vi "Measurement UI.vi"() -> ()   [LabVIEW 2021, in "Line Regulation_PMIC.lvlib"]
uses:
  Line Regulation_PMIC.lvlib
panel:
  in  "MeasGraphs":T1(tab)
  out "LineRegulationGraph(V/V)":T2(graph)
  out "LineRegulationGraph(%)":T3(graph)
  out "Maximum load voltage deviation":dbl
  out "Minimum load voltage deviation":dbl
  out "Maximum load voltage":dbl
  out "Minimum load voltage":dbl
  out "Load voltage deviation":dbl[](array[numeric])
  out "Load voltages":dbl[](array[numeric])
  out "Source voltages":dbl[](array[numeric])
  in  "Source resource name":string caption="RESOURCE NAME"
  in  "Load resource name":string caption="RESOURCE NAME"
  out "MeasTable":string[][](table)
  in  "Load sense":i32(ring)=1009 caption="SENSE" items=["Local"=1008, "Remote"=1009]
  in  "Source sense":i32(ring)=1009 caption="SENSE" items=["Local"=1008, "Remote"=1009]
  out "Status":string
  in  "ELOADResourceName":refnum<k15> caption="RESOURCE NAME"
  in  "PPSResourceName":refnum<k15> caption="RESOURCE NAME"
  in  "Source sweep type":string(combo)="Logarithmic" caption="SWEEP TYPE"
  in  "DUT setup time":dbl=1.0 caption="DUT SETUP TIME" format="%#_6ps"
  in  "Source stop voltage":dbl=20.0 caption="STOP VOLTAGE" format="%#_6pV"
  in  "Source start voltage":dbl=6.0 caption="START VOLTAGE" format="%#_6pV"
  in  "Source voltage sweep points/points per decade":i32=10 caption="PTS/PTS PER DECADE"
  in  "Aperture time":dbl=0.005 caption="APERTURE TIME" format="%#_6ps"
  in  "Source delay":dbl=0.005 caption="SOURCE DELAY" format="%#_6ps"
  in  "Load current level":dbl=1.0 caption="CURRENT  LEVEL" format="%#_6pA"
  in  "Load voltage limit range":dbl=6.0 caption="VOLTAGE LIMIT RANGE" format="%#_6pV"
  in  "Source current limit":dbl=25.0 caption="CURRENT LIMIT" format="%#_6pA"
  in  "Source maximum power":dbl=300.0 caption="MAXIMUM POWER" format="%#_6pW"
  in  "Load configuration":string="Load configuration"
  in  "Source configuration":string="Source configuration"
  in  "Measurement settings":string="Measurement settings"
  in  "Nominal output voltage":dbl=3.3 caption="NOMINAL OUTPUT VOLTAGE" format="%#_6pV"
  in  "Mode of operation":T4(ring)=enum."Perform measurement" caption="MODE OF OPERATION"
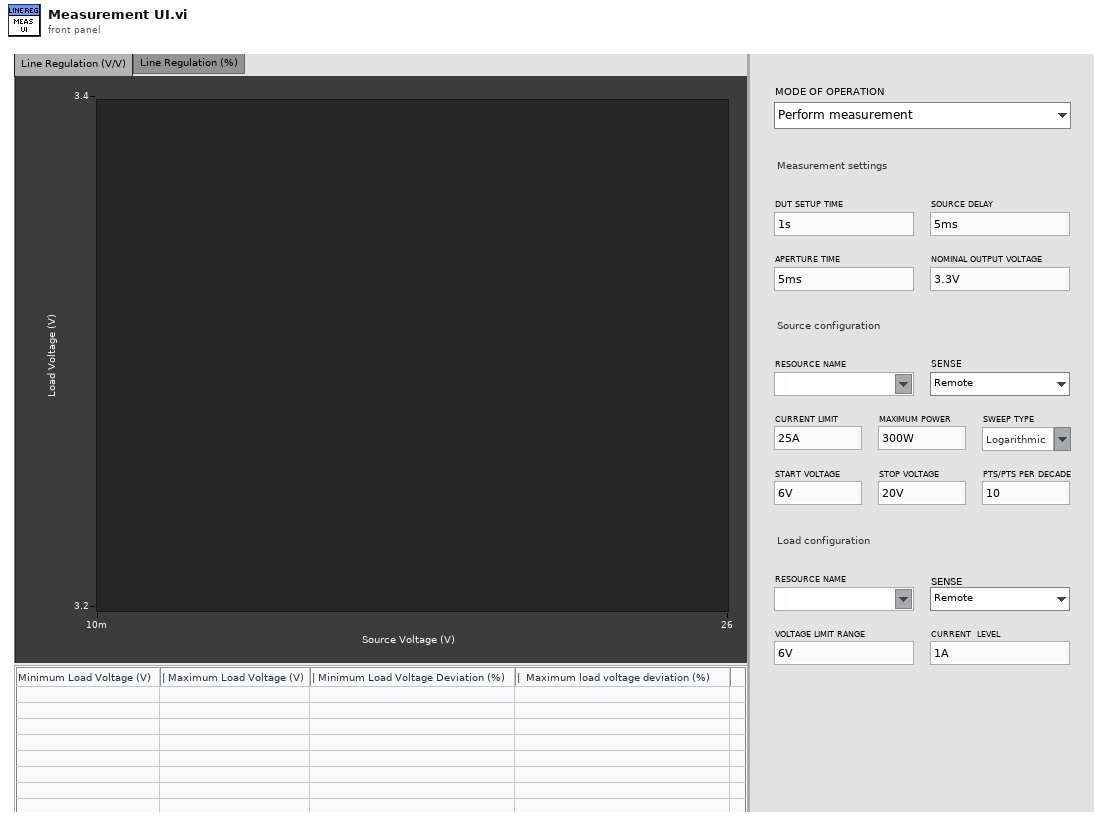
[diagram p1: front panel]
types:
  T1 = enum32{"Line Regulation (V/V)", "Line Regulation (%)", "Hidden Controls"}
  T2 = cluster{"Source voltages":dbl[], "Load voltages":dbl[]}
  T3 = cluster{"Source voltages":dbl[], "Load voltage deviation":dbl[]}
  T4 = enum32{"Power on the DUT", "Perform measurement", "Power off the DUT"}
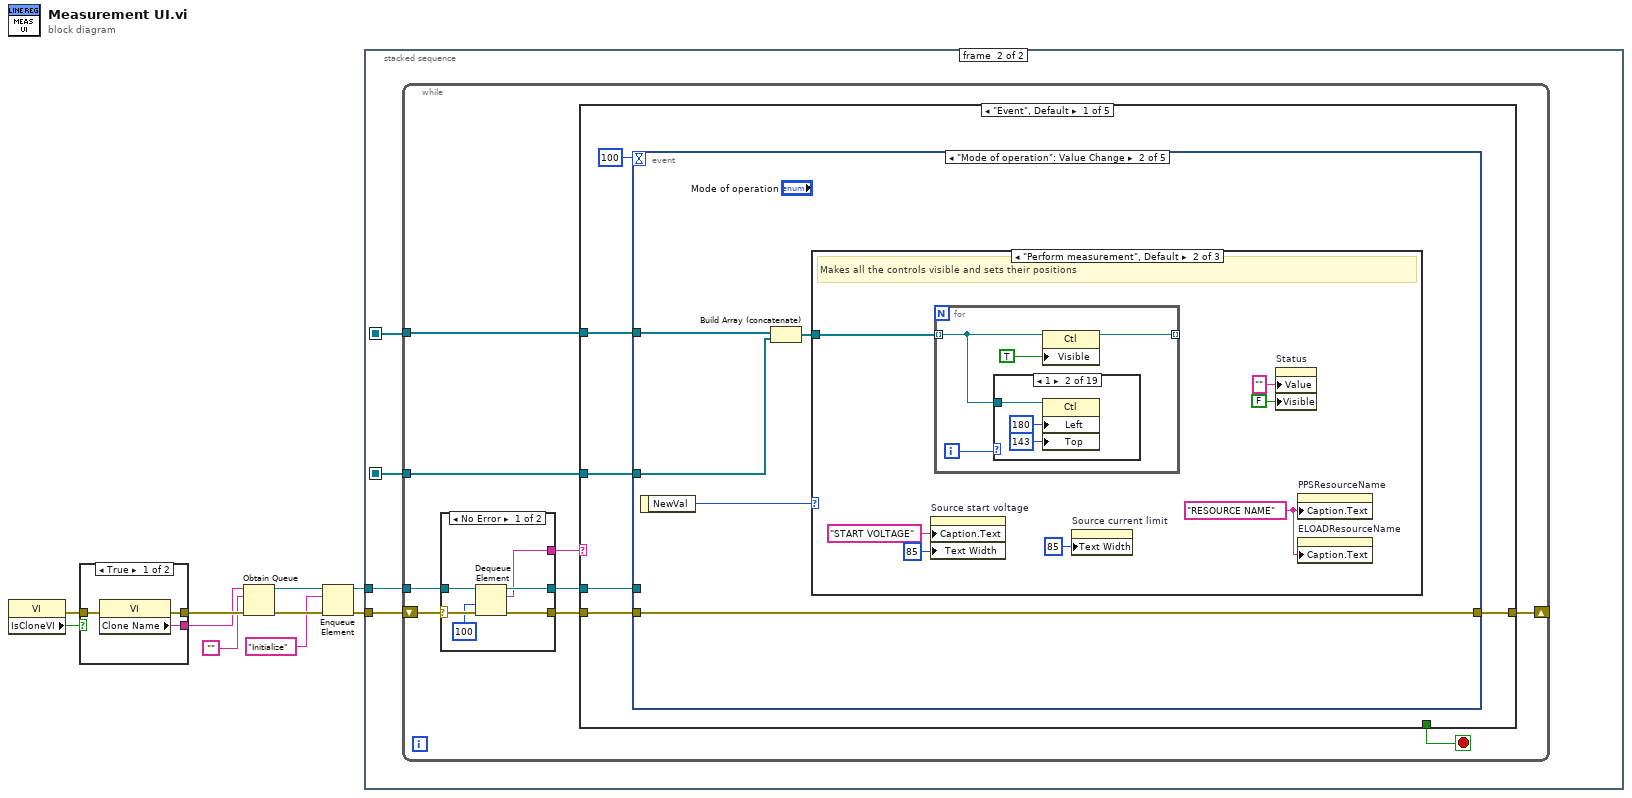
[diagram p0: block diagram]
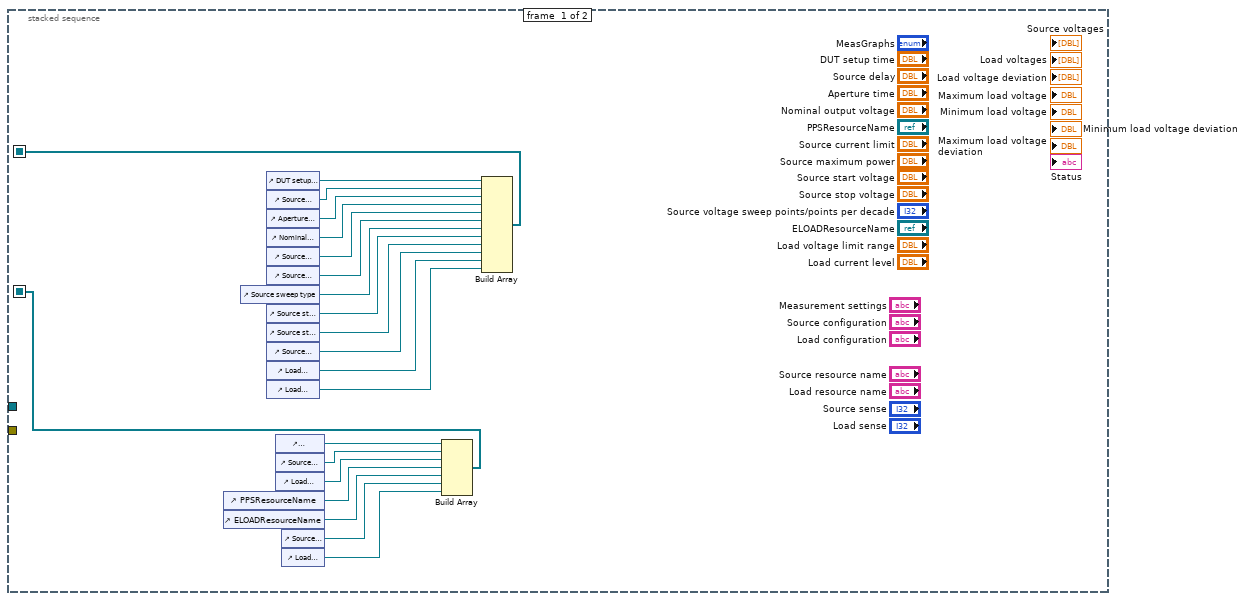
[diagram p2: hidden frame]
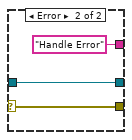
[diagram p3: hidden frame]
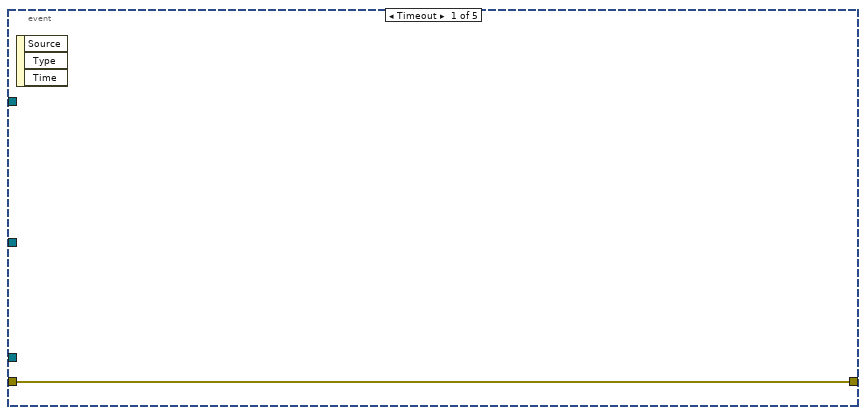
[diagram p4: hidden frame]
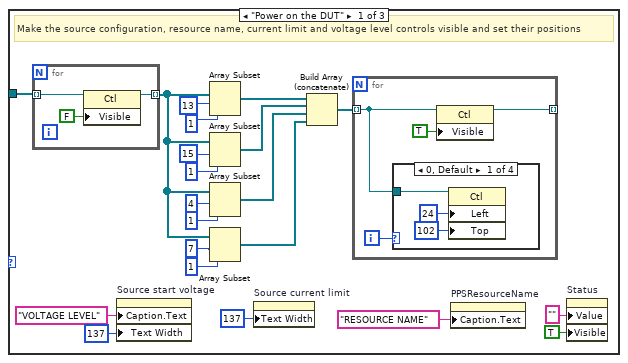
[diagram p5: hidden frame]
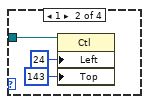
[diagram p6: hidden frame]
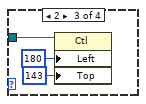
[diagram p7: hidden frame]
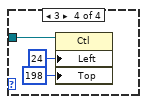
[diagram p8: hidden frame]
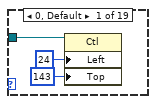
[diagram p9: hidden frame]
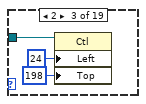
[diagram p10: hidden frame]
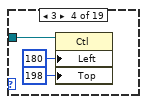
[diagram p11: hidden frame]
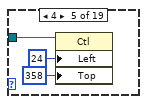
[diagram p12: hidden frame]
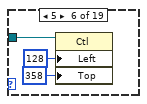
[diagram p13: hidden frame]
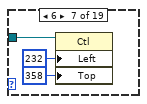
[diagram p14: hidden frame]
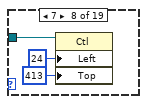
[diagram p15: hidden frame]
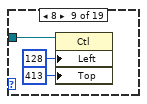
[diagram p16: hidden frame]
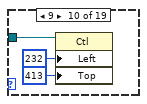
[diagram p17: hidden frame]
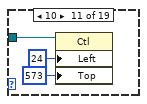
[diagram p18: hidden frame]
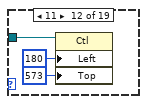
[diagram p19: hidden frame]
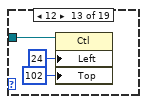
[diagram p20: hidden frame]
diagram:
  n1 = property class="VI"() -> (error out=w1:errorcluster, "IsCloneVI"=w2:bool)  [unwired: 2 in, 1 out]
  n2 = case shown="True" w2 {
    tunnel: [w13 w16] -> w10
    tunnel: [w12 w15] -> w9
    tunnel: w1 -> [w11 w14]
    frame True {
      n3 = property class="VI"(error in=w11) -> (error out=w13:errorcluster, "Clone Name"=w12:string)  [unwired: 1 in, 1 out]
    }
    frame False {
      n4 = property class="VI"(error in=w14) -> (error out=w16:errorcluster, "Name"=w15:string)  [unwired: 1 in, 1 out]
    }
  }
  n5 = Obtain Queue(name (unnamed)=w9, element data type="", error in (no error)=w10) -> (queue out=w6:refnum<queue>, error out=w8:errorcluster)  [unwired: 2 in, 1 out]
  n6 = Enqueue Element(queue=w6, element="Initialize", error in (no error)=w8) -> (queue out=w5:refnum<queue>, error out=w7:errorcluster)  [unwired: 1 in, 1 out]
  n7 = stacked-sequence {
    seq-local: [w20 _] -> [_ w39]
    seq-local: [w19 _] -> [_ w38]
    tunnel: w7 -> [_ w41]
    tunnel: w5 -> [_ w40]
    frame #0 {
      n8 = control-ref of="PPSResourceName"() -> (w23:refnum<vi>)
      n9 = control-ref of="ELOADResourceName"() -> (w22:refnum<vi>)
      n10 = control-ref of="Source sweep type"() -> (w21:refnum<vi>)
      n11 = control-ref of="DUT setup time"() -> (w37:refnum<vi>)
      n12 = control-ref of="Source delay"() -> (w36:refnum<vi>)
      n13 = control-ref of="Aperture time"() -> (w35:refnum<vi>)
      n14 = control-ref of="Nominal output voltage"() -> (w27:refnum<vi>)
      n15 = control-ref of="Source current limit"() -> (w34:refnum<vi>)
      n16 = control-ref of="Source maximum power"() -> (w33:refnum<vi>)
      n17 = control-ref of="Source start voltage"() -> (w32:refnum<vi>)
      n18 = control-ref of="Source stop voltage"() -> (w31:refnum<vi>)
      n19 = control-ref of="Source voltage sweep points/points per decade"() -> (w30:refnum<vi>)
      n20 = control-ref of="Load voltage limit range"() -> (w29:refnum<vi>)
      n21 = control-ref of="Load current level"() -> (w28:refnum<vi>)
      n22 = control-ref of="Measurement settings"() -> (w26:refnum<vi>)
      n23 = control-ref of="Source configuration"() -> (w24:refnum<vi>)
      n24 = control-ref of="Load configuration"() -> (w25:refnum<vi>)
      n25 = control-ref of="Source sense"() -> (w18:refnum<vi>)
      n26 = control-ref of="Load sense"() -> (w17:refnum<vi>)
      n27 = Build Array(w26, w24, w25, w23, w22, w18, w17) -> (w19:refnum<vi>[])
      n28 = Build Array(w37, w36, w35, w27, w34, w33, w21, w32, w31, w30, w29, w28) -> (w20:refnum<vi>[])
    }
    frame #1 {
      n29 = while {
        shift-right: [w45] -> _
        shift-left: w41 -> [w50]
        tunnel: w40 -> [w48]
        tunnel: w39 -> [w43]
        tunnel: w38 -> [w42]
        stop <- w44 stop-if-true
        n30 = case shown="No Error" w50 {
          selector: w50 -> [w56 w59]
          tunnel: [w55 w59] -> w49
          tunnel: w48 -> [w54 w58]
          tunnel: [w53 w58] -> w47
          tunnel: [w52 "Handle Error"] -> w46
          frame No Error {
            n31 = Dequeue Element(queue=w54, timeout in ms (-1)=100, error in (no error)=w56) -> (queue out=w53:refnum<queue>, element=w52:string, error out=w55:errorcluster)  [unwired: 1 out]
          }
          frame Error {
          }
        }
        n32 = case shown="\"Event\", Default" w46 {
          tunnel: w49 -> [w64 w216 w243 w257 w258]
          tunnel: w47 -> [w62 _ _ w255 _]
          tunnel: [w65 w216 w243 w249 w258] -> w45
          tunnel: [_ _ _ TRUE _] -> w44
          tunnel: w43 -> [w61 _ _ w248 _]
          tunnel: w42 -> [w60 _ _ w247 _]
          frame "Event", Default {
            n33 = event shown="[1] \"Mode of operation\": Value Change" {
              selector: _ -> [_ _ _ _ _]
              dyn-events: _ -> [_ _ _ _ _]
              timeout: 100 -> [_ _ _ _ _]
              tunnel: [w66 w67 w202 w204 w208] -> w65
              tunnel: w64 -> [w66 w67 w202 w204 w209]
              tunnel: w62 -> [_ _ _ _ w207]
              tunnel: w61 -> [_ w68 _ _ _]
              tunnel: w60 -> [_ w70 _ _ _]
              event Timeout {
                n34 = event-data() -> ()  [unwired: 1 in, 3 out]
              }
              event "Mode of operation": Value Change {
                n35 = event-data() -> ("NewVal"=w71:T4)  [unwired: 1 in]
                n36 = Build Array (concatenate)(w68, w70) -> (w69:refnum<vi>[])
                n37 = case shown="\"Perform measurement\", Default" w71 {
                  tunnel: w69 -> [w84 w118 w185]
                  frame "Power on the DUT" {
                    # "Make the source configuration, resource name, current limit and voltage level controls visible and set their positions"
                    n38 = for {
                      tunnel: w84 -> [w95] mode=indexing
                      tunnel: [w93] -> w81 mode=indexing
                      n39 = property class="Ctl"(reference=w95, "Visible"=FALSE) -> (reference out=w93:refnum<vi>)  [unwired: 1 in, 1 out]
                    }
                    n40 = property on="Source start voltage" class="DigNum (strict)"("Caption.Text"="VOLTAGE LEVEL", "Text Width"=u32 137) -> ()  [unwired: 2 in, 2 out]
                    n41 = Array Subset(array=w81, index=13 ("length"), length=1 ("index")) -> (w83:refnum<vi>[])
                    n42 = Array Subset(array=w81, index=15 ("length"), length=1 ("index")) -> (w82:refnum<vi>[])
                    n43 = Array Subset(array=w81, index=4 ("length"), length=1 ("index")) -> (w80:refnum<vi>[])
                    n44 = Array Subset(array=w81, index=7 ("length"), length=1 ("index")) -> (w78:refnum<vi>[])
                    n45 = property on="Source current limit" class="DigNum (strict)"("Text Width"=u32 137) -> ()  [unwired: 2 in, 2 out]
                    n46 = Build Array (concatenate)(w83, w82, w80, w78) -> (w79:refnum<vi>[])
                    n47 = for {
                      tunnel: [w98] -> _ mode=indexing
                      tunnel: w79 -> [w96] mode=indexing
                      i -> [w97]
                      n48 = case shown="0, Default" w97 {
                        tunnel: w96 -> [w102 w105 w108 w111]
                        frame 0, Default {
                          n49 = property class="Ctl"(reference=w102, "Left"=24 ("Position:Left"), "Top"=102 ("Position:Top")) -> ()  [unwired: 1 in, 2 out]
                        }
                        frame 1 {
                          n50 = property class="Ctl"(reference=w105, "Left"=24 ("Position:Left"), "Top"=143 ("Position:Top")) -> ()  [unwired: 1 in, 2 out]
                        }
                        frame 2 {
                          n51 = property class="Ctl"(reference=w108, "Left"=180 ("Position:Left"), "Top"=143 ("Position:Top")) -> ()  [unwired: 1 in, 2 out]
                        }
                        frame 3 {
                          n52 = property class="Ctl"(reference=w111, "Left"=24 ("Position:Left"), "Top"=198 ("Position:Top")) -> ()  [unwired: 1 in, 2 out]
                        }
                      }
                      n53 = property class="Ctl"(reference=w96, "Visible"=TRUE) -> (reference out=w98:refnum<vi>)  [unwired: 1 in, 1 out]
                    }
                    n54 = property on="PPSResourceName" class="IVIName"("Caption.Text"="RESOURCE NAME") -> ()  [unwired: 2 in, 2 out]
                    n55 = property on="Status" class="Str"("Value"="" ("Operation"), "Visible"=TRUE) -> ()  [unwired: 2 in, 2 out]
                  }
                  frame "Perform measurement", Default {
                    w116 = "RESOURCE NAME" ("Caption.Text")
                    # "Makes all the controls visible and sets their positions"
                    n56 = property on="Source start voltage" class="DigNum (strict)"("Caption.Text"="START VOLTAGE", "Text Width"=u32 85) -> ()  [unwired: 2 in, 2 out]
                    n57 = for {
                      tunnel: w118 -> [w119] mode=indexing
                      tunnel: [w121] -> _ mode=indexing
                      i -> [w120]
                      n58 = case shown="1" w120 {
                        tunnel: w119 -> [w125 w128 w131 w134 w137 w140 w143 w146 w149 w152 w155 w158 w161 w164 w167 w170 w173 w174 w177]
                        frame 0, Default {
                          n59 = property class="Ctl"(reference=w125, "Left"=24 ("Position:Left"), "Top"=143 ("Position:Top")) -> ()  [unwired: 1 in, 2 out]
                        }
                        frame 1 {
                          n60 = property class="Ctl"(reference=w128, "Left"=180 ("Position:Left"), "Top"=143 ("Position:Top")) -> ()  [unwired: 1 in, 2 out]
                        }
                        frame 2 {
                          n61 = property class="Ctl"(reference=w131, "Left"=24 ("Position:Left"), "Top"=198 ("Position:Top")) -> ()  [unwired: 1 in, 2 out]
                        }
                        frame 3 {
                          n62 = property class="Ctl"(reference=w134, "Left"=180 ("Position:Left"), "Top"=198 ("Position:Top")) -> ()  [unwired: 1 in, 2 out]
                        }
                        frame 4 {
                          n63 = property class="Ctl"(reference=w137, "Left"=24 ("Position:Left"), "Top"=358 ("Position:Top")) -> ()  [unwired: 1 in, 2 out]
                        }
                        frame 5 {
                          n64 = property class="Ctl"(reference=w140, "Left"=128 ("Position:Left"), "Top"=358 ("Position:Top")) -> ()  [unwired: 1 in, 2 out]
                        }
                        frame 6 {
                          n65 = property class="Ctl"(reference=w143, "Left"=232 ("Position:Left"), "Top"=358 ("Position:Top")) -> ()  [unwired: 1 in, 2 out]
                        }
                        frame 7 {
                          n66 = property class="Ctl"(reference=w146, "Left"=24 ("Position:Left"), "Top"=413 ("Position:Top")) -> ()  [unwired: 1 in, 2 out]
                        }
                        frame 8 {
                          n67 = property class="Ctl"(reference=w149, "Left"=128 ("Position:Left"), "Top"=413 ("Position:Top")) -> ()  [unwired: 1 in, 2 out]
                        }
                        frame 9 {
                          n68 = property class="Ctl"(reference=w152, "Left"=232 ("Position:Left"), "Top"=413 ("Position:Top")) -> ()  [unwired: 1 in, 2 out]
                        }
                        frame 10 {
                          n69 = property class="Ctl"(reference=w155, "Left"=24 ("Position:Left"), "Top"=573 ("Position:Top")) -> ()  [unwired: 1 in, 2 out]
                        }
                        frame 11 {
                          n70 = property class="Ctl"(reference=w158, "Left"=180 ("Position:Left"), "Top"=573 ("Position:Top")) -> ()  [unwired: 1 in, 2 out]
                        }
                        frame 12 {
                          n71 = property class="Ctl"(reference=w161, "Left"=24 ("Position:Left"), "Top"=102 ("Position:Top")) -> ()  [unwired: 1 in, 2 out]
                        }
                        frame 13 {
                          n72 = property class="Ctl"(reference=w164, "Left"=24 ("Position:Left"), "Top"=262 ("Position:Top")) -> ()  [unwired: 1 in, 2 out]
                        }
                        frame 14 {
                          n73 = property class="Ctl"(reference=w167, "Left"=24 ("Position:Left"), "Top"=477 ("Position:Top")) -> ()  [unwired: 1 in, 2 out]
                        }
                        frame 15 {
                          n74 = property class="Ctl"(reference=w170, "Left"=24 ("Position:Left"), "Top"=303 ("Position:Top")) -> ()  [unwired: 1 in, 2 out]
                        }
                        frame 16 {
                          n75 = property class="Ctl"(reference=w173, "Left"=24 ("Position:Left"), "Top"=518 ("Position:Top")) -> ()  [unwired: 1 in, 2 out]
                        }
                        frame 17 {
                          n76 = property class="Ctl"(reference=w174, "Left"=180 ("Position:Left"), "Top"=303 ("Position:Top")) -> ()  [unwired: 1 in, 2 out]
                        }
                        frame 18 {
                          n77 = property class="Ctl"(reference=w177, "Left"=180 ("Position:Left"), "Top"=518 ("Position:Top")) -> ()  [unwired: 1 in, 2 out]
                        }
                      }
                      n78 = property class="Ctl"(reference=w119, "Visible"=TRUE) -> (reference out=w121:refnum<vi>)  [unwired: 1 in, 1 out]
                    }
                    n79 = property on="Source current limit" class="DigNum (strict)"("Text Width"=u32 85) -> ()  [unwired: 2 in, 2 out]
                    n80 = property on="Status" class="Str"("Value"="" ("Status"), "Visible"=FALSE) -> ()  [unwired: 2 in, 2 out]
                    n81 = property on="PPSResourceName" class="IVIName"("Caption.Text"=w116) -> ()  [unwired: 2 in, 2 out]
                    n82 = property on="ELOADResourceName" class="IVIName"("Caption.Text"=w116) -> ()  [unwired: 2 in, 2 out]
                  }
                  frame "Power off the DUT" {
                    # "Makes only the Source and Load Resource Name controls visible and sets their positions"
                    n83 = for {
                      tunnel: w185 -> [w190] mode=indexing
                      tunnel: [w189] -> w184 mode=indexing
                      n84 = property class="Ctl"(reference=w190, "Visible"=FALSE) -> (reference out=w189:refnum<vi>)  [unwired: 1 in, 1 out]
                    }
                    n85 = Array Subset(array=w184, index=15 ("length"), length=2 ("index")) -> (w186:refnum<vi>[])
                    n86 = property on="PPSResourceName" class="IVIName"("Caption.Text"="SOURCE RESOURCE NAME") -> ()  [unwired: 2 in, 2 out]
                    n87 = property on="ELOADResourceName" class="IVIName"("Caption.Text"="LOAD RESOURCE NAME") -> ()  [unwired: 2 in, 2 out]
                    n88 = for {
                      tunnel: w186 -> [w192] mode=indexing
                      tunnel: [w194] -> _ mode=indexing
                      i -> [w193]
                      n89 = case shown="0, Default" w193 {
                        tunnel: w192 -> [w198 w201]
                        frame 0, Default {
                          n90 = property class="Ctl"(reference=w198, "Left"=24 ("Position:Left"), "Top"=102 ("Position:Top")) -> ()  [unwired: 1 in, 2 out]
                        }
                        frame 1 {
                          n91 = property class="Ctl"(reference=w201, "Left"=24 ("Position:Left"), "Top"=157 ("Position:Top")) -> ()  [unwired: 1 in, 2 out]
                        }
                      }
                      n92 = property class="Ctl"(reference=w192, "Visible"=TRUE) -> (reference out=w194:refnum<vi>)  [unwired: 1 in, 1 out]
                    }
                    n93 = property on="Status" class="Str"("Value"="" ("Operation"), "Visible"=TRUE) -> ()  [unwired: 2 in, 2 out]
                  }
                }
              }
              event "PPSResourceName": Value Change {
                n94 = event-data() -> ()  [unwired: 1 in, 1 out]
                n95 = property on="PPSResourceName" class="IVIName"() -> ("Value"=w203:refnum<k15>)  [unwired: 2 in, 2 out]
                n96 = property on="Source resource name" class="Str"("Value"=w203) -> ()  [unwired: 2 in, 2 out]
              }
              event "ELOADResourceName": Value Change {
                n97 = event-data() -> ()  [unwired: 1 in, 1 out]
                n98 = property on="ELOADResourceName" class="IVIName"() -> ("Value"=w205:refnum<k15>)  [unwired: 2 in, 2 out]
                n99 = property on="Load resource name" class="Str"("Value"=w205) -> ()  [unwired: 2 in, 2 out]
              }
              event Panel Close? {
                n100 = event-data() -> ()  [unwired: 1 in, 1 out]
                n101 = Enqueue Element(queue=w207, element="Exit", error in (no error)=w209) -> (error out=w208:errorcluster)  [unwired: 1 in, 2 out]
                n102 = event-data("Discard?"=TRUE) -> ()  [unwired: 1 in, 1 out]
              }
            }
          }
          frame "Initialize" {
            w215 = "<Select Device>"
            n103 = control-ref of="LineRegulationGraph(V/V)"() -> (w214:refnum<vi>)
            n104 = control-ref of="LineRegulationGraph(%)"() -> (w213:refnum<vi>)
            n105 = Build Array(w214, w213) -> (w212:refnum<vi>[])
            n106 = for {
              tunnel: w212 -> [w217] mode=indexing
              n107 = property class="XYGraph (strict)"(reference=w217, "ActPaletteTool"=2 ("Palette:Active Tool")) -> ()  [unwired: 1 in, 2 out]
            }
            n108 = property on="PPSResourceName" class="IVIName"("Value"=w215) -> ()  [unwired: 2 in, 2 out]
            n109 = property on="ELOADResourceName" class="IVIName"("Value"=w215) -> ()  [unwired: 2 in, 2 out]
            n110 = property on="Status" class="Str"("Visible"=FALSE) -> ()  [unwired: 2 in, 2 out]
          }
          frame "Post UI Update" {
            w228 = "%.3f" ("initial string")
            w227 = "|   " ("initial string")
            # "This case will be triggered, after framework updates the User interface with result values."
            n111 = control-ref of="LineRegulationGraph(V/V)"() -> (w233:refnum<vi>)
            n112 = control-ref of="LineRegulationGraph(%)"() -> (w232:refnum<vi>)
            n113 = local read "Maximum load voltage deviation"() -> (w219:dbl)
            n114 = local read "Minimum load voltage deviation"() -> (w220:dbl)
            n115 = Not Equal?(x="Linear", y="Source sweep type") -> (x != y?=w236:bool)
            n116 = Build Array(w233, w232) -> (w231:refnum<vi>[])
            n117 = local read "Maximum load voltage"() -> (w221:dbl)
            n118 = local read "Minimum load voltage"() -> (w230:dbl)
            n119 = Boolean To (0,1)(Boolean=w236) -> (0, 1=w235:i16)
            n120 = for {
              tunnel: w231 -> [w245] mode=indexing
              tunnel: w235 -> [w244]
              n121 = property class="XYGraph (strict)"(reference=w245, "XScale.Mapping Mode"=w244) -> ()  [unwired: 1 in, 2 out]
            }
            n122 = local read "Load voltage deviation"() -> (w241:dbl[])
            n123 = local read "Source voltages"() -> (w240:dbl[])
            n124 = local read "Load voltages"() -> (w242:dbl[])
            n125 = Format Into String(format string=w228, w230) -> (resulting string=w229:string)  [unwired: 2 in, 1 out]
            n126 = Format Into String(format string=w228, initial string=w227, w221) -> (resulting string=w226:string)  [unwired: 1 in, 1 out]
            n127 = Format Into String(format string=w228, initial string=w227, w220) -> (resulting string=w225:string)  [unwired: 1 in, 1 out]
            n128 = Format Into String(format string=w228, initial string=w227, w219) -> (resulting string=w224:string)  [unwired: 1 in, 1 out]
            n129 = Bundle("Source voltages"=w240, "Load voltages"=w242) -> (→"LineRegulationGraph(V/V)":T2)  [unwired: 1 in]
            n130 = Bundle("Source voltages"=w240, "Load voltage deviation"=w241) -> (→"LineRegulationGraph(%)":T3)  [unwired: 1 in]
            n131 = Build Array(w229, w226, w225, w224) -> (w223:string[])
            n132 = Build Array(w223) -> (→"MeasTable":string[][])
          }
          frame "Exit" {
            # "This case is triggered to close the User Interface from framework"
            n133 = Build Array (concatenate)(w248, w247) -> (w246:refnum<vi>[])
            n134 = Close Reference(reference=w246) -> (error out=w251:errorcluster)  [unwired: 1 in]
            n135 = Flush Queue(queue=w255, error in (no error)=w257) -> (queue out=w254:refnum<queue>, error out=w253:errorcluster)  [unwired: 1 out]
            n136 = Release Queue(queue=w254, force destroy? (F)=TRUE, error in (no error)=w253) -> (error out=w250:errorcluster)  [unwired: 2 out]
            n137 = Merge Errors(w251, w250) -> (w249:errorcluster)
          }
          frame "Handle Error" {
          }
        }
      }
    }
  }
